vi "run tests.vi"() -> (3 "No error?":bool)   [LabVIEW 2013]
panel:
  out "Tests":T1(array[cluster])
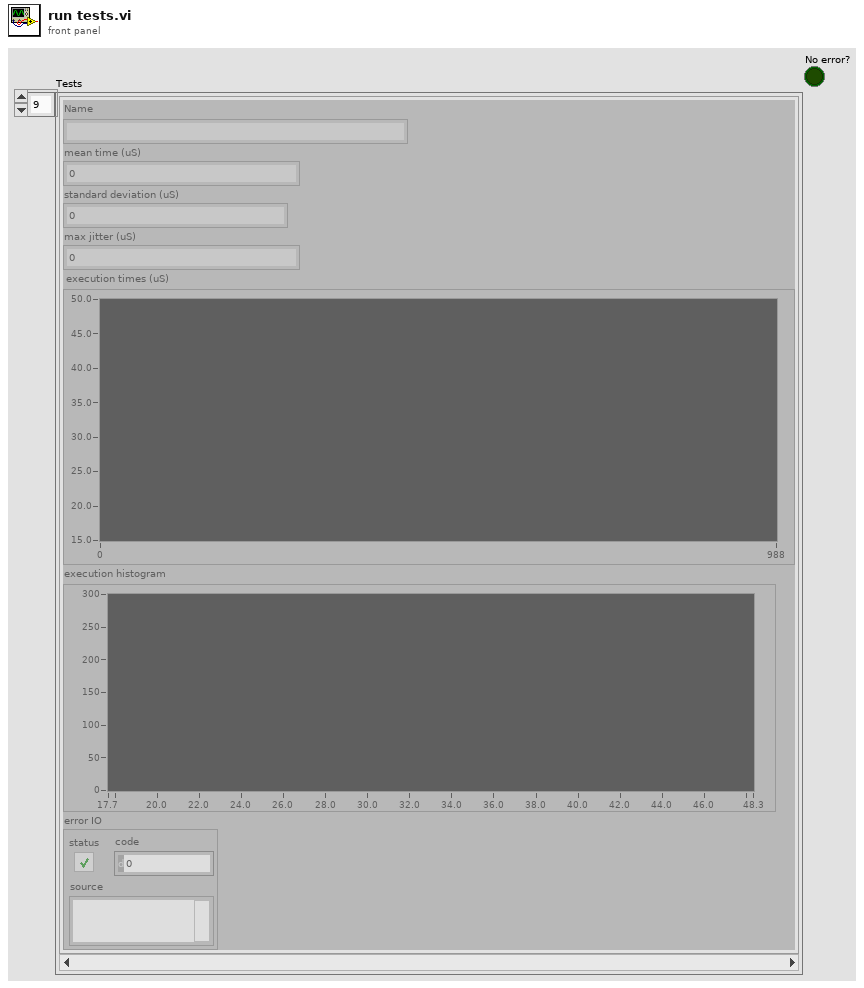
[diagram p1: front panel]
types:
  T1 = cluster{"Name":string, "mean time (uS)":dbl, "standard deviation (uS)":dbl, "max jitter (uS)":dbl, "execution times (uS)":dbl[], "execution histogram":cluster{"X Values":dbl[], "Histogram: h(x)":i32[]}, "error IO":errorcluster}[]
  T2 = cluster{"X Values":dbl[], "Histogram: h(x)":i32[]}
  T3 = cluster{"name":string, "mean time (uS)":dbl, "standard deviation (uS)":dbl, "max jitter (uS)":dbl, "execution times (uS)":dbl[], "execution histogram":cluster{"X Values":dbl[], "Histogram: h(x)":i32[]}, "error IO":errorcluster}
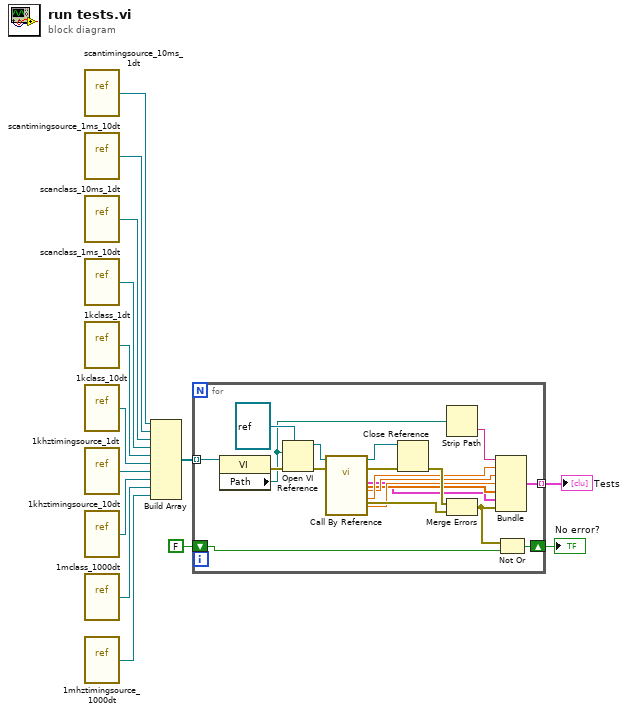
[diagram p0: block diagram]
diagram:
  n1 = vi-ref "scantimingsource_10ms_1dt.vi"() -> (w14:refnum<vi>)
  n2 = vi-ref "scantimingsource_1ms_10dt.vi"() -> (w13:refnum<vi>)
  n3 = vi-ref "scanclass_10ms_1dt.vi"() -> (w12:refnum<vi>)
  n4 = vi-ref "scanclass_1ms_10dt.vi"() -> (w11:refnum<vi>)
  n5 = vi-ref "1kclass_1dt.vi"() -> (w8:refnum<vi>)
  n6 = vi-ref "1kclass_10dt.vi"() -> (w7:refnum<vi>)
  n7 = vi-ref "1khztimingsource_1dt.vi"() -> (w6:refnum<vi>)
  n8 = vi-ref "1khztimingsource_10dt.vi"() -> (w5:refnum<vi>)
  n9 = vi-ref "1mclass_1000dt.vi"() -> (w4:refnum<vi>)
  n10 = vi-ref "1mhztimingsource_1000dt.vi"() -> (w3:refnum<vi>)
  n11 = Build Array(w14, w13, w12, w11, w8, w7, w6, w5, w4, w3) -> (w10:refnum<vi>[])
  n12 = for {
    tunnel: w10 -> [w34] mode=indexing
    tunnel: [w20] -> w9 mode=indexing
    shift-right: [w16] -> w1
    shift-left: FALSE -> [w15]
    n13 = property class="VI"(reference=w34) -> (error out=w33:errorcluster, "Path"=w19:path)  [unwired: 1 in, 1 out]
    n14 = Open VI Reference(type specifier VI Refnum (for type only)=refnum<vi> refnum, vi path=w19, error in (no error)=w33) -> (vi reference=w31:refnum<vi>, error out=w32:errorcluster)  [unwired: 3 in]
    n15 = call-by-ref "?"(reference=w31, error in=w32) -> (reference out=w28:refnum<vi>, error out=w29:errorcluster, "max jitter (uS)"=w23:dbl, "mean time (uS)"=w25:dbl, "standard deviation (uS)"=w24:dbl, "execution histogram"=w21:T2, "Error"=w26:errorcluster, "execution times (uS)"=w22:dbl[])  [unwired: 6 in]
    n16 = Close Reference(reference=w28, error in (no error)=w29) -> (error out=w27:errorcluster)
    n17 = Strip Path(path=w19) -> (name=w18:string)  [unwired: 1 out]
    n18 = Merge Errors(w27, w26) -> (w17:errorcluster)
    n19 = Bundle("name"=w18, "mean time (uS)"=w25, "standard deviation (uS)"=w24, "max jitter (uS)"=w23, "execution times (uS)"=w22, "execution histogram"=w21, "error IO"=w17) -> (w20:T3)  [unwired: 1 in]
    n20 = Not Or(1:w15, 2:w17) -> (0:w16:bool)
  }
  "Tests" <- w9
  "No error?" <- w1
